vi "10-send&receive-arrays.vi"() -> ()   [LabVIEW 2018, in "LV2Julia_examples.lvlib"]
uses:
  LV2Julia_examples.lvlib
  LV2Julia_core/VIs/Server or client state.ctl
  LV2Julia_core/VIs/detailed error info.ctl
  LV2Julia_core/VIs/StackFrame.ctl
  LV2Julia_core/VIs/Numeric Types enum.ctl
  array 123D sizes.ctl
  LV2Julia_core/VIs/Commands.ctl
  LV2Julia_core/VIs/ZMQ timeouts.ctl
  19565153-6e23-41a7-814d-e58de81dde5a.vi
  5ef99b4f-9bfc-4a0d-a8a0-74b261859f3d.vi
  388a3b2a-e541-4e37-ba3b-5749cefc77c1.vi
  e91abbe1-2489-4f0d-9743-379a6a4cbf4d.vi
  19565153-6e23-41a7-814d-e58de81dde5a.vi/f8b41fa0-dc66-4675-9ab2-69071d8e11b4.vi
  <vilib>/Utility/High Resolution Relative Seconds.vi
  388a3b2a-e541-4e37-ba3b-5749cefc77c1.vi/942dbbfe-0971-4a07-8155-21945c62de4e.vi
  19565153-6e23-41a7-814d-e58de81dde5a.vi/f8b41fa0-dc66-4675-9ab2-69071d8e11b4.vi/e6eaab0a-a73c-4bc6-9fc3-66bb032cf3db.vi
  19565153-6e23-41a7-814d-e58de81dde5a.vi/f8b41fa0-dc66-4675-9ab2-69071d8e11b4.vi/89c65089-1604-4a02-9ccd-ea27dc7a2819.vi
  19565153-6e23-41a7-814d-e58de81dde5a.vi/f8b41fa0-dc66-4675-9ab2-69071d8e11b4.vi/542429cb-615c-43e9-bb26-5fc81b0b2517.vi
  388a3b2a-e541-4e37-ba3b-5749cefc77c1.vi/942dbbfe-0971-4a07-8155-21945c62de4e.vi/0f446f5b-a377-42cc-a7f3-40c12ec29588.vi
  388a3b2a-e541-4e37-ba3b-5749cefc77c1.vi/942dbbfe-0971-4a07-8155-21945c62de4e.vi/5a652f4c-4df5-4f4b-9a5e-c969a1bae96c.vi
  388a3b2a-e541-4e37-ba3b-5749cefc77c1.vi/942dbbfe-0971-4a07-8155-21945c62de4e.vi/1240bcb9-7ce4-487b-a9f5-f5568576f487.vi
  LV2Julia_core/VIs/jl-scripts path.vi
  LV2Julia_core/VIs/check ID validity.vi
  LV2Julia_core/VIs/bindata_descr to JSON.vi
  LV2Julia_core/VIs/check cluster field names.vi
  LV2Julia_core/VIs/concat JSON.vi
  LV2Julia_core/VIs/build request.vi
  LV2Julia_core/VIs/Parse server response.vi
  LV2Julia_core/VIs/log jl exceptions.vi
  LV2Julia_core/LV2Julia_core.lvlib
panel:
  out "ZMQ timeout":bool
  out "Julia script file path":path
  out "temporary script path":path
  in  "execution control pages":enum32{"Start&stop", "go - test", "error"}(tab)
  in  "go":bool caption="go (Julia Server started externally)"
  in  "Start with Julia":bool caption="Start Julia Server and go"
  in  "ZMQ endpoint":string="tcp://127.0.0.1:5555"
  out "Jl Server state":T1
  out "numarray 3D":cdb[][][](array[numeric])
  out "numarray 2D":cdb[][](array[numeric])
  out "numarray 1D":cdb[](array[numeric]) format="%.1f"
  out "numeric type":T2
  out "arr dimension":i32
  out "all arrays OK":bool
  out "arrs equal":bool
  out "array sizes":T3
  out "el_type":string
  out "arsize":i32[](array[numeric])
  out "data flattening delta t":dbl
  out "flattening ms/MB":dbl format="%#.2f"
  out "Zmq&Julia delta t":dbl
  out "Zmq&JUlia ms/MB":dbl format="%#.2f"
  out "data unflattening delta t":dbl
  out "unflattening ms/MB":dbl format="%#.2f"
  in  "stop VI":bool caption="stop this VI only"
  in  "stop both":bool caption="stop both this VI and Julia Server"
  in  "returnarrs":bool=TRUE
  in  "log2(arrsize)":u32=7 min=5
  in  "cycle min time (s)":sgl min=0 step=0.2
  in  "next":bool
  out "warm up":bool
  in  "test extent":enum32{"all types", "spec type"}(tab)
  in  "arr type":T2
  in  "dims":cluster{"1D":bool, "2D":bool, "3D":bool}
  in  "rounds":u32=1 min=1
  out "detailed error info":T4
  out "current error":errorcluster
  out "final error":errorcluster
  out "short err code":u8
  # "tcp://127.0.0.1:5555 \nfor local Julia Server\n\nFor a Julia Server running on a separate computer,  you probably must use an IPv4 address in numeric form (not a DNS name) - see https://stackoverflow.com/questions/6024003/why-doesnt-zeromq-work-on-localhost.\n\nFor instructions how to properly start the corresponding Julia script, see \n05-on_external_server.jl file in the jl-scripts folder.\n\nThe ZMQ endpoint control only used if Julia Server is not being started by this VI."
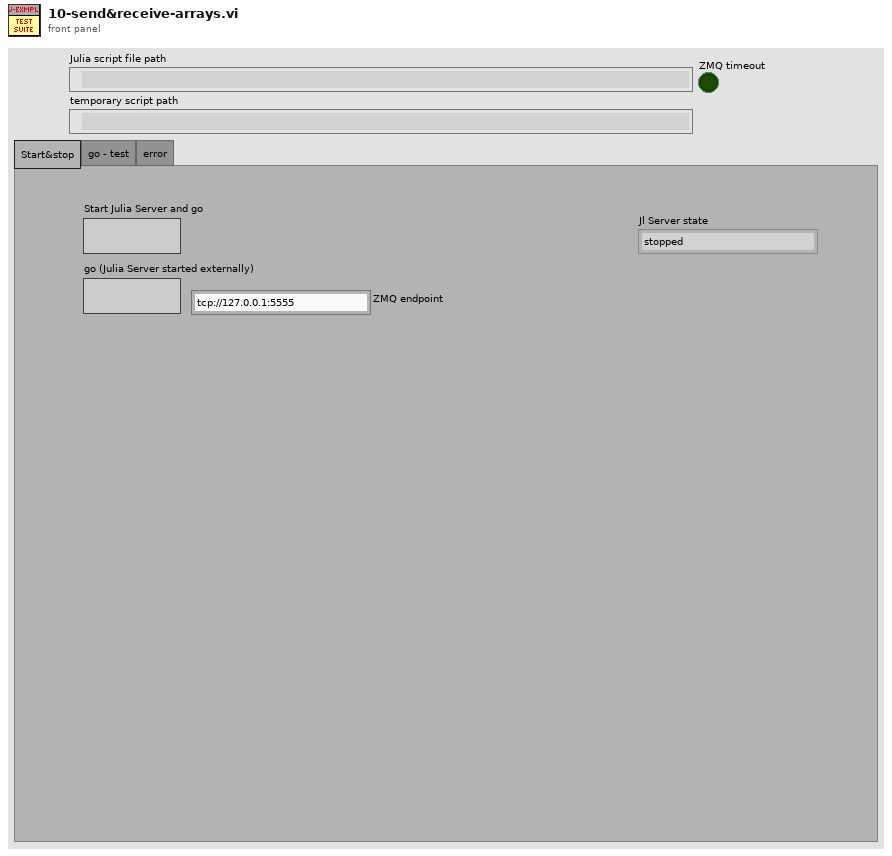
[diagram p1: front panel]
types:
  T1 = typedef "LV2Julia_core.lvlib/Server or client state.ctl" = enum16{"stopped", "running", "unknown"}
  T2 = typedef "LV2Julia_core.lvlib/Numeric Types enum.ctl" = enum16{"SGL", "DBL", "I8", "I16", "I32", "I64", "U8", "U16", "U32", "U64", "CSGL", "CDBL", "boolean"}
  T3 = typedef "LV2Julia_examples.lvlib/array 123D sizes.ctl" = cluster{"s1":i32, "s2":i32[], "s3":i32[]}
  T4 = typedef "LV2Julia_core.lvlib/detailed error info.ctl" = cluster{"exception_or_info":string, "trace":T5[]}
  T5 = typedef "LV2Julia_core.lvlib/StackFrame.ctl" = cluster{"frame_summary":string, "func":string, "linfo":string, "file":string, "line":i32, "pointer":u64, "from_c":bool, "inlined":bool}
  T6 = typedef "LV2Julia_core.lvlib/ZMQ timeouts.ctl" = cluster{"SNDTIMEO":i32, "RCVTIMEO":i32}
  T7 = typedef "LV2Julia_core.lvlib/Commands.ctl" = enum16{"Start Jl-server & Init LV-client", "Send request & Get response ", "Stop Jl-server & Cleanup LV-client", "Cleanup LV-client", "Start Jl-server", "Stop Jl-server", "Init LV-Client", "Cleanup LV-Client", "(not allowed)", "Set LV Client state", "Set Jl Server state", "set ZMQ timeout", "read ZMQ timeout", "read-out state"}
  T8 = typedef "LV2Julia_core.lvlib/Bindata&description.ctl" = cluster{"bindata_descr":T9[], "bindata":u8[]}
  T9 = typedef "LV2Julia_core.lvlib/Bindata description.ctl" = cluster{"nofbytes":i32, "numtype":string, "start":i32, "arrdims":i32[], "kwarg_name":string, "category":string}
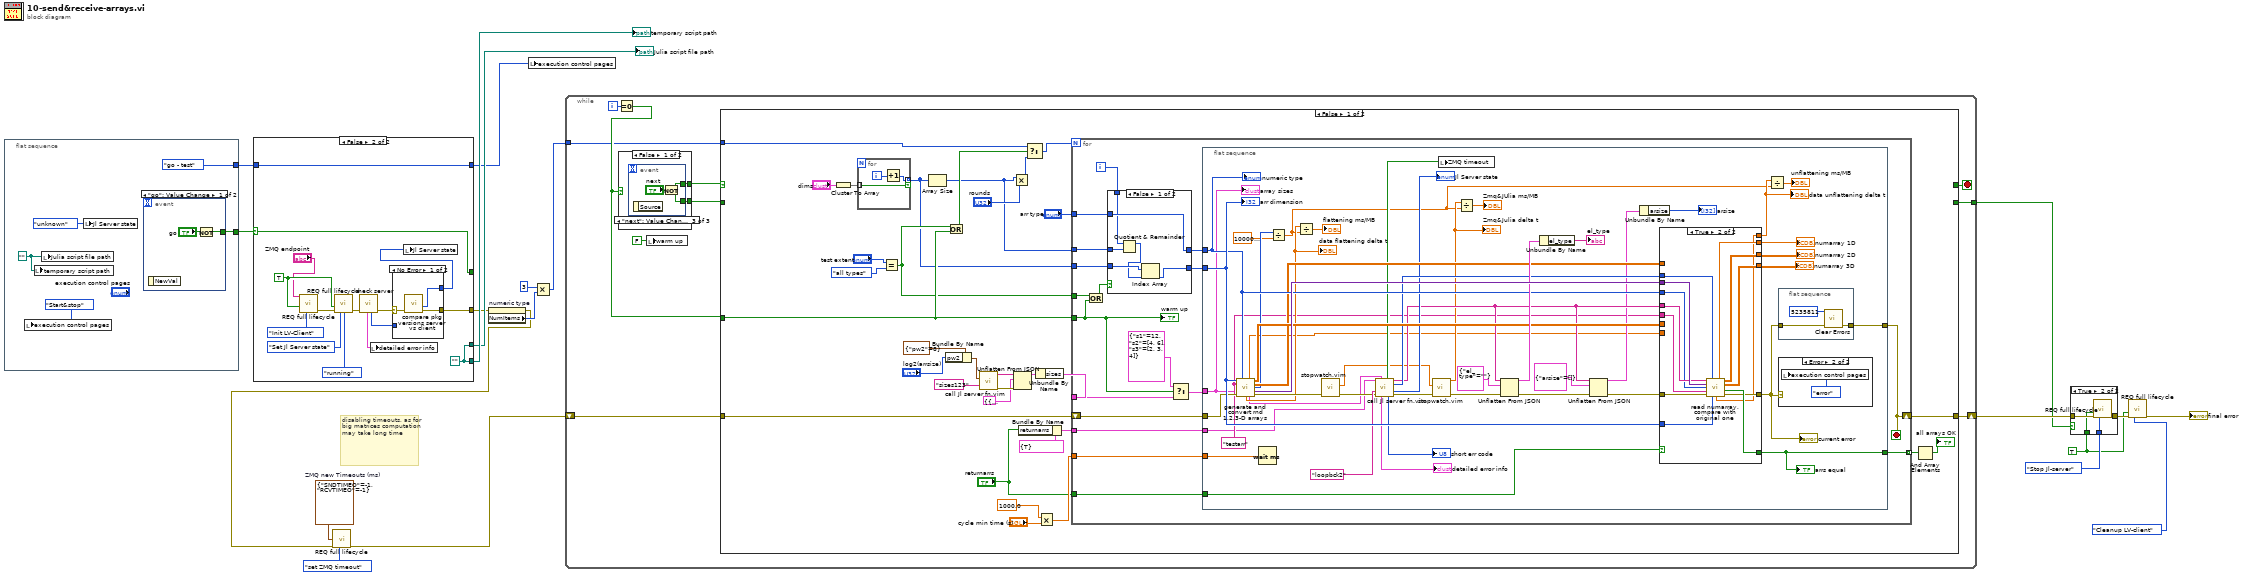
[diagram p0: block diagram]
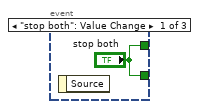
[diagram p2: hidden frame]
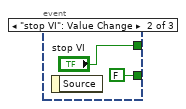
[diagram p3: hidden frame]
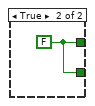
[diagram p4: hidden frame]
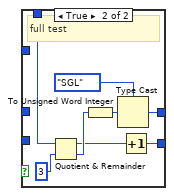
[diagram p5: hidden frame]
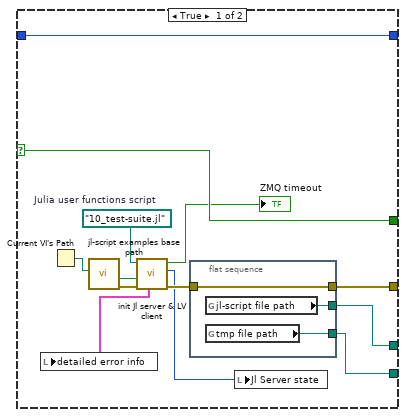
[diagram p9: hidden frame]
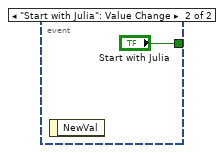
[diagram p11: hidden frame]
diagram:
  w3 = T6 {"SNDTIMEO"=-1, "RCVTIMEO"=-1}  # ZMQ new Timeouts (ms)
  w16 = TRUE ("Force command")
  # "disabling timeouts, as for big matrices computation may take long time"
  n1 = flat-sequence {
    tunnel: [w23] -> w12
    tunnel: [enum32{"Start&stop", "go - test", "error"}."go - test" ("execution control pages")] -> w7
    frame #0 {
      w24 = path ""
      n2 = local write "execution control pages"(enum32{"Start&stop", "go - test", "error"}."Start&stop" ("execution control pages")) -> ()
      n3 = local write "temporary script path"(w24) -> ()
      n4 = local write "Julia script file path"(w24) -> ()
      n5 = local write "Jl Server state"(Server_or_client_state."unknown" ("Jl Server state out")) -> ()
      n6 = event shown="[0] \"go\": Value Change" {
        selector: _ -> [_ _]
        dyn-events: _ -> [_ _]
        timeout: _ -> [_ _]
        tunnel: [w26 "Start with Julia"] -> w23
        event "go": Value Change {
          n7 = event-data() -> ()  [unwired: 1 in, 1 out]
          n8 = Not(x="go") -> (.not. x?=w26:bool)
        }
        event "Start with Julia": Value Change {
          n9 = event-data() -> ()  [unwired: 1 in, 1 out]
        }
      }
    }
  }
  n10 = case shown="False" w12 {
    selector: w12 -> [w41 w55]
    tunnel: [w40 w50] -> w9
    tunnel: [w41 w55] -> _
    tunnel: [w39 w52] -> w10
    tunnel: [w38 w52] -> w11
    tunnel: [w30 w46] -> w8
    tunnel: w7 -> [w30 w46]
    frame True {
      w32 = path "10_test-suite.jl"  # Julia user functions script
      n11 = Current VI's Path() -> (path=w36:path)
      n12 = call "jl-script examples base path.vi"("calling example VI path"=w36) -> ("error out"=w35:errorcluster, "jl-script-examples base path"=w34:path)  [unwired: 9 in]
      n13 = call "init Jl server & LV client.vi"("error in (no error)"=w35, "Base path (not a path)"=w34, "Julia user functions script"=w32) -> ("error out"=w37:errorcluster, "Jl Server state out"=w33:T1, "timeout?"=→"ZMQ timeout":bool, "detailed error info"=w29:T4)  [unwired: 3 in, 2 out]
      n14 = local write "detailed error info"(w29) -> ()
      n15 = flat-sequence {
        tunnel: [w44] -> w40
        tunnel: w37 -> [w44]
        tunnel: [w43] -> w39
        tunnel: [w42] -> w38
        frame #0 {
          n16 = global read "jl-scripts path.vi" "jl-script file path"() -> (w43:path)
          n17 = global read "jl-scripts path.vi" "tmp file path"() -> (w42:path)
        }
      }
      n18 = local write "Jl Server state"(w33) -> ()
    }
    frame False {
      w52 = path ""
      w57 = TRUE ("Force command")
      n19 = call "REQ full lifecycle.vi"("ZMQ endpoint"="ZMQ endpoint", "Force command"=w57, "command"=Commands."Init LV-Client") -> ("error out"=w54:errorcluster)  [unwired: 6 in, 6 out]
      n20 = call "REQ full lifecycle.vi"("Force command"=w57, "error in"=w54, "command"=Commands."Set Jl Server state", "Jl Server state in"=Server_or_client_state."running") -> ("error out"=w53:errorcluster)  [unwired: 5 in, 6 out]
      n21 = call "check server.vi"("error in"=w53) -> ("error out"=w51:errorcluster, "Jl Server state out"=w49:T1, "detailed error info"=w45:T4)  [unwired: 6 in, 2 out]
      n22 = local write "detailed error info"(w45) -> ()
      n23 = case shown="No Error" w51 {
        selector: w51 -> [w62 w64]
        tunnel: [w61 w64] -> w50
        tunnel: [w60 w63] -> w47
        tunnel: w49 -> [_ w63]
        frame No Error {
          n24 = call "compare pkg versions server vs client.vi"("error in (no error)"=w62) -> ("error out"=w61:errorcluster, "Jl Server state out"=w60:T1)  [unwired: 5 in, 4 out]
        }
        frame Error {
        }
      }
      n25 = local write "Jl Server state"(w47) -> ()
    }
  }
  "temporary script path" <- w11
  "Julia script file path" <- w10
  n26 = property on="numeric type" class="Enum (strict)"(error in=w9) -> (error out=w1:errorcluster, "NumItems"=w15:u32)  [unwired: 1 in, 1 out]
  n27 = call "REQ full lifecycle.vi"("ZMQ new Timeouts in"=w3, "error in"=w1, "command"=Commands."set ZMQ timeout") -> ("error out"=w2:errorcluster)  [unwired: 6 in, 6 out]
  n28 = local write "execution control pages"(w8) -> ()
  n29 = Multiply(x=u32 3, y=w15) -> (x*y=w13:u32)
  n30 = while {
    tunnel: w13 -> [w65]
    shift-right: [w74] -> w6
    shift-left: w2 -> [w73]
    tunnel: [w71] -> w5
    i -> [w68]
    stop <- w69 stop-if-true
    n31 = Equal To 0?(x=w68) -> (x = 0?=w66:bool)
    n32 = case shown="False" w66 {
      tunnel: [w76 w82] -> w72
      tunnel: [w75 w82] -> w70
      frame False {
        n33 = event shown="[2] \"next\": Value Change" {
          selector: _ -> [_ _ _]
          dyn-events: _ -> [_ _ _]
          timeout: _ -> [_ _ _]
          tunnel: ["stop both" "stop VI" w80] -> w75
          tunnel: ["stop both" FALSE ("stop both this VI and Julia Server") w80] -> w76
          event "stop both": Value Change {
            n34 = event-data() -> ()  [unwired: 1 in, 1 out]
          }
          event "stop VI": Value Change {
            n35 = event-data() -> ()  [unwired: 1 in, 1 out]
          }
          event "next": Value Change {
            n36 = event-data() -> ()  [unwired: 1 in, 1 out]
            n37 = Not(x="next") -> (.not. x?=w80:bool)
          }
        }
      }
      frame True {
        w82 = FALSE ("stop this VI only")
      }
    }
    n38 = local write "warm up"(FALSE ("warm up")) -> ()
    n39 = case shown="False" w70 {
      selector: w70 -> [_ w221]
      tunnel: [w115 w220] -> w74
      tunnel: w73 -> [w114 w220]
      tunnel: [_ w222] -> w71
      tunnel: w72 -> [_ w222]
      tunnel: [_ w221] -> w69
      tunnel: w66 -> [w107 _]
      tunnel: w65 -> [w109 _]
      frame False {
        n40 = Cluster To Array(cluster="dims") -> (array=w88:bool[])
        n41 = for {
          tunnel: w88 -> [w116] mode=indexing
          tunnel: [w117] -> w83 mode=indexing if=w116
          i -> [w118]
          n42 = Increment(x=w118) -> (x+1=w117:i32)
        }
        n43 = Equal?(x="test extent", y=enum32{"all types", "spec type"}."all types" ("test extent")) -> (x = y?=w86:bool)
        n44 = Array Size(array=w83) -> (size(s)=w84:i32)
        n45 = Bundle By Name(cluster=cluster{"pw2":u32} {"pw2"=8}, "pw2"="log2(arrsize)") -> (w102:cluster{"pw2":u32})
        n46 = Or(x=w86, y=w107) -> (x .or. y?=w87:bool)
        n47 = call "call Jl server fn.vim"("Arguments 2"=w102, "fun2call"="sizes123") -> ("JSON received"=w105:string, "error out"=w106:errorcluster)  [unwired: 7 in, 5 out]
        n48 = Multiply(x=w84, y="rounds") -> (x*y=w85:u32)
        n49 = Unflatten From JSON(JSON string=w105, type and defaults=cluster{"sizes":T3} {"sizes"={"s1"=0, "s2"=[], "s3"=[]}}, error in (no error)=w106) -> (value=w104:cluster{"sizes":T3})  [unwired: 4 in, 1 out]
        n50 = Bundle By Name(cluster=cluster{"returnarrs":bool} {"returnarrs"=TRUE}, "returnarrs"="returnarrs") -> (w94:cluster{"returnarrs":bool})
        n51 = Select(t=w109, s=w87, f=w85) -> (s? t:f=w108:u32)
        n52 = Unbundle By Name(w104) -> ("sizes"=w98:T3)
        n53 = Multiply(x=sgl 1000.0, y="cycle min time (s)") -> (x*y=w95:sgl)
        n54 = for {
          N: w108 -> [_]
          tunnel: [w129] -> w113 mode=indexing
          shift-right: [w134] -> w115
          shift-left: w114 -> [w135]
          tunnel: w94 -> [w131]
          tunnel: "returnarrs" -> [w132]
          tunnel: w98 -> [w126]
          tunnel: w95 -> [w130]
          tunnel: w107 -> [w124]
          tunnel: "arr type" -> [w123]
          tunnel: w86 -> [w121]
          tunnel: w84 -> [w120]
          tunnel: w83 -> [w119]
          i -> [w128]
          stop <- w134 stop-if-true
          n55 = Or(x=w121, y=w124) -> (x .or. y?=w122:bool)
          n56 = case shown="False" w122 {
            tunnel: [w137 w145] -> w136
            tunnel: [w142 w144] -> w133
            tunnel: w128 -> [w140 w143]
            tunnel: w123 -> [w142 _]
            tunnel: w120 -> [w141 _]
            tunnel: w119 -> [w139 _]
            frame False {
              n57 = Quotient & Remainder(x=w140, y=w141) -> (x-y*floor(x/y)=w138:i32)  [unwired: 1 out]
              n58 = Index Array(array=w139, index=w138) -> (element=w137:i32)
            }
            frame True {
              # "full test"
              n59 = Quotient & Remainder(x=w143, y=3) -> (x-y*floor(x/y)=w146:i32, floor(x/y)=w147:i32)
              n60 = To Unsigned Word Integer(number=w147) -> (unsigned 16bit integer=w148:u16)
              n61 = Type Cast(type=Numeric_Types_enum."SGL" ("numeric type const"), x=w148) -> (*(type *) &x=w144:T2)
              n62 = Increment(x=w146) -> (x+1=w145:i32)
            }
          }
          n63 = Select(t=T3 {"s1"=12, "s2"=[4, 6], "s3"=[2, 3, 4]} ("f"), s=w124, f=w126) -> (s? t:f=w127:T3)
          n64 = flat-sequence {
            tunnel: w136 -> [w196]
            tunnel: w135 -> [w195]
            tunnel: [w194] -> w134
            tunnel: w133 -> [w190]
            tunnel: w132 -> [w187]
            tunnel: w131 -> [w154]
            tunnel: w127 -> [w155]
            tunnel: w130 -> [w178]
            tunnel: [w159] -> w129
            frame #0 {
              w156 = "testarr" ("Tag")
              n65 = call "generate and convert rnd 1,2,3-D arrays.vi"("dims"=w196, "numeric type const"=w190, "Tag"=w156, "sizes"=w155, "error in (no error)"=w195) -> ("Array 1D"=w151:cdb[], "Array 2D"=w186:cdb[][], "Array 3D"=w185:cdb[][][], "bytes"=w160:i32, "array as variant"=w198:variant, "delta t (s)"=w166:dbl, "Bindata & descr out"=w153:T8, "error out"=w170:errorcluster)  [unwired: 1 in, 2 out]
              "data flattening delta t" <- w166
              n66 = Wait (ms)(milliseconds to wait=w178) -> ()  [unwired: 1 out]
              n67 = Divide(x=w160, y=1000000000.0) -> (x/y=w157:dbl)
              n68 = Divide(x=w166, y=w157) -> (x/y=→"flattening ms/MB":dbl)
              n69 = call "stopwatch.vim"("anything in"=w170) -> ("copy of anything out"=w169:errorcluster, "current timepoint"=w171:dbl)  [unwired: 8 in, 1 out]
              n70 = call "call Jl server fn.vim"("Arguments 1"=w154, "Bindata & descr in"=w153, "fun2call"="loopbck2", "error in (no error)"=w169) -> ("timeout?"=w179:bool, "JSON received"=w175:string, "binary data received"=w182:u8[], "Jl Server state out"=→"Jl Server state":T1, "detailed error info"=→"detailed error info":T4, "return code"=→"short err code":u8, "error out"=w168:errorcluster)  [unwired: 5 in]
              n71 = call "stopwatch.vim"("anything in"=w168, "prev timepoint (0)"=w171) -> ("copy of anything out"=w167:errorcluster, "delta t (s)"=w163:dbl)  [unwired: 7 in, 1 out]
              "Zmq&Julia delta t" <- w163
              n72 = local write "ZMQ timeout"(w179) -> ()
              n73 = Divide(x=w163, y=w157) -> (x/y=→"Zmq&JUlia ms/MB":dbl)
              n74 = Unflatten From JSON(JSON string=w175, type and defaults=cluster{"el_type":string} {"el_type"=""} ("parsed response"), error in (no error)=w167) -> (value=w193:cluster{"el_type":string}, error out=w177:errorcluster)  [unwired: 4 in]
              n75 = Unbundle By Name(w193) -> ("el_type"=→"el_type":string)
              n76 = Unflatten From JSON(JSON string=w175, type and defaults=cluster{"arsize":i32[]} {"arsize"=[]} ("parsed response"), error in (no error)=w177) -> (value=w173:cluster{"arsize":i32[]}, error out=w176:errorcluster)  [unwired: 4 in]
              n77 = Unbundle By Name(w173) -> ("arsize"=→"arsize":i32[])
              n78 = case shown="True" w187 {
                tunnel: w182 -> [_ w215]
                tunnel: [w201 w214] -> w152
                tunnel: w198 -> [_ w213]
                tunnel: [w199 w212] -> w197
                tunnel: [_ w211] -> w159
                tunnel: w196 -> [_ w210]
                tunnel: w176 -> [w202 w209]
                tunnel: w175 -> [_ w208]
                tunnel: w156 -> [_ w207]
                tunnel: w190 -> [_ w206]
                tunnel: [w200 w205] -> w189
                tunnel: [w202 w204] -> w188
                tunnel: w151 -> [w201 _]
                tunnel: w186 -> [w200 _]
                tunnel: w185 -> [w199 _]
                tunnel: [_ w203] -> w161
                frame False {
                }
                frame True {
                  n79 = call "read numarray, compare with original one.vi"("JSON in"=w208, "binary data in"=w215, "array as variant in"=w213, "numeric type"=w206, "kwarg_name"=w207, "error in (no error)"=w209, "dims"=w210) -> ("numarray 1D"=w214:cdb[], "numarray 2D"=w205:cdb[][], "numarray 3D"=w212:cdb[][][], "arrays are equal"=w211:bool, "delta t (s)"=w203:dbl, "error out"=w204:errorcluster)  [unwired: 1 in, 2 out]
                }
              }
              "numarray 1D" <- w152
              "arrs equal" <- w159
              "numarray 2D" <- w189
              "numarray 3D" <- w197
              "current error" <- w188
              "data unflattening delta t" <- w161
              n80 = Divide(x=w161, y=w157) -> (x/y=→"unflattening ms/MB":dbl)
              n81 = flat-sequence {
                tunnel: w188 -> [w219]
                tunnel: [w218] -> w194
                frame #0 {
                  n82 = call <vilib>:"Clear Errors.vi"("error in (no error)"=w219, "specific error code to clear (0: all)"=5235811) -> ("error out"=w218:errorcluster)  [unwired: 4 in, 1 out]
                }
              }
              n83 = case shown="Error" w188 {
                frame No Error {
                }
                frame Error {
                  n84 = local write "execution control pages"(enum32{"Start&stop", "go - test", "error"}."error" ("execution control pages")) -> ()
                }
              }
              "numeric type" <- w190
              "arr dimension" <- w196
              "array sizes" <- w155
            }
          }
          "warm up" <- w124
        }
        n85 = And Array Elements(Boolean array=w113) -> (logical AND=→"all arrays OK":bool)
      }
      frame True {
        # "stop"
      }
    }
  }
  n86 = case shown="True" w5 {
    tunnel: w6 -> [w223 w227]
    tunnel: Commands."Stop Jl-server" ("command") -> [_ w226]
    tunnel: [w223 w225] -> w19
    tunnel: w16 -> [_ w224]
    frame False {
    }
    frame True {
      n87 = call "REQ full lifecycle.vi"("Force command"=w224, "error in"=w227, "command"=w226) -> ("error out"=w225:errorcluster)  [unwired: 6 in, 6 out]
    }
  }
  n88 = call "REQ full lifecycle.vi"("Force command"=w16, "error in"=w19, "command"=Commands."Cleanup LV-client") -> ("error out"=→"final error":errorcluster)  [unwired: 6 in, 6 out]
